vi "Check Close.vi"(8 "error in (no error)":errorcluster, 11 "Module in":refnum<class "Module.lvclass">) -> (0 "error out":errorcluster, 2 "Stop":bool, 3 "Module out":refnum<class "Module.lvclass">)   [LabVIEW 2020, in "Volatus.lvlib" / "Module.lvclass"]
uses:
  Module.lvclass
  Module.lvclass/Module.ctl
  Event Level.ctl
  State.ctl
  8a5c0d25-5ba7-4b78-9c46-4168992e23e7.vi
  Volatus.lvlib
panel:
  out "Module ID":string
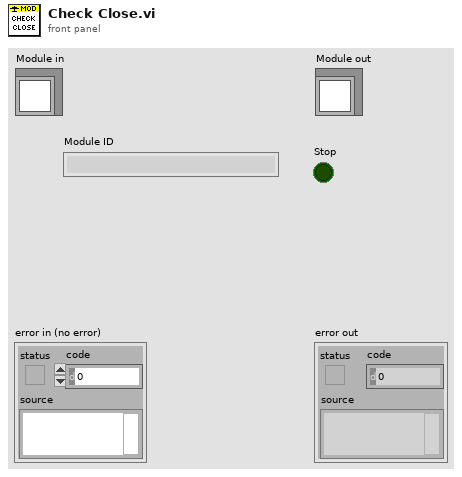
[diagram p1: front panel]
types:
  T1 = typedef "Volatus.lvlib/Module.lvclass/State.ctl" = enum16{"Unknown", "Launched", "Starting", "Running", "Stopping", "Stopped", "Error - Starting", "Error - Run", "Error - Stopping"}
  T2 = typedef "Volatus.lvlib/Event Level.ctl" = enum16{"Debug", "Info", "Warning", "Error"}
  T3 = typedef "Volatus.lvlib/Module Status.ctl" = cluster{"MessageQ":refnum<class "MessageQ.lvclass">, "State":T1, "Hierarchy":string[], "Forwarded":bool}
  T4 = cluster{"MsgQ":refnum<class "MessageQ.lvclass">, "Status":T3}[]
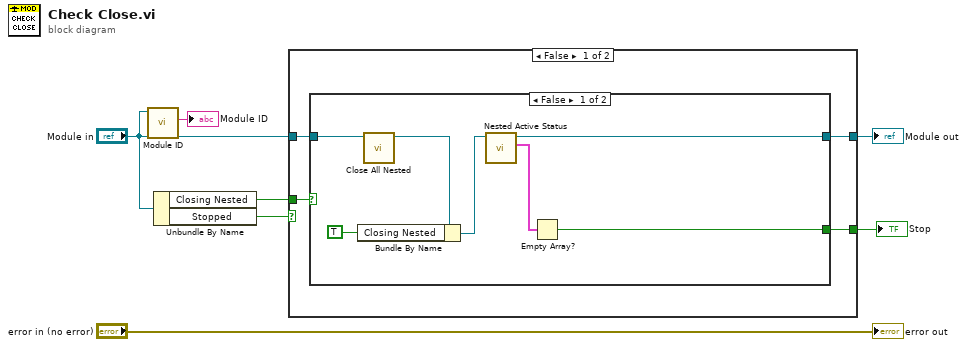
[diagram p0: block diagram]
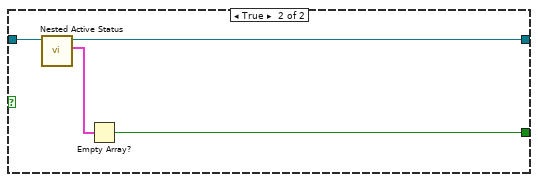
[diagram p2: hidden frame]
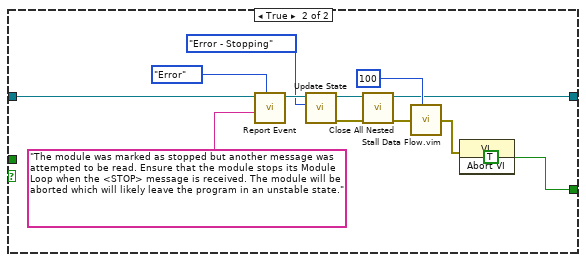
[diagram p3: hidden frame]
diagram:
  n1 = call-dynamic "Module ID.vi"("Module in"="Module in") -> ("Module ID"=→"Module ID":string)  [unwired: 10 in]
  n2 = Unbundle By Name("Module in") -> ("Closing Nested"=w7:bool, "Stopped"=w3:bool)
  n3 = case shown="False" w3 {
    tunnel: "Module in" -> [w11 w34]
    tunnel: w7 -> [w10 _]
    tunnel: [w9 w23] -> w6
    tunnel: [w8 TRUE] -> w4
    frame False {
      n4 = case shown="False" w10 {
        tunnel: w11 -> [w18 w22]
        tunnel: [w12 w21] -> w9
        tunnel: [w13 w19] -> w8
        frame False {
          n5 = call "Close All Nested.vi"("Module in"=w18) -> ("Module out"=w17:refnum<class "Module.lvclass">)  [unwired: 9 in, 1 out]
          n6 = Bundle By Name(cluster=w17, "Closing Nested"=TRUE) -> (w16:refnum<class "Module.lvclass">)
          n7 = call "Nested Active Status.vi"("Module in"=w16) -> ("Active Nested"=w14:T4, "Module out"=w12:refnum<class "Module.lvclass">)  [unwired: 7 in, 2 out]
          n8 = Empty Array?(array=w14) -> (empty?=w13:bool)
        }
        frame True {
          n9 = call "Nested Active Status.vi"("Module in"=w22) -> ("Active Nested"=w20:T4, "Module out"=w21:refnum<class "Module.lvclass">)  [unwired: 7 in, 2 out]
          n10 = Empty Array?(array=w20) -> (empty?=w19:bool)
        }
      }
    }
    frame True {
      n11 = call "Report Event.vi"("Level (Info)"=Event_Level."Error", "Message"="The module was marked as stopped but another message was attempted to be read. Ensure that the module stops its Module Loop when the <STOP> message is received. The module will be aborted which will likely leave the program in an unstable state.", "Module in"=w34) -> ("Module out"=w31:refnum<class "Module.lvclass">)  [unwired: 7 in, 1 out]
      n12 = call "Update State.vi"("State"=State."Error - Stopping", "Module in"=w31) -> ("error out"=w27:errorcluster, "Module out"=w24:refnum<class "Module.lvclass">)  [unwired: 8 in]
      n13 = call "Close All Nested.vi"("error in (no error)"=w27, "Module in"=w24) -> ("error out"=w25:errorcluster, "Module out"=w23:refnum<class "Module.lvclass">)  [unwired: 8 in]
      n14 = call "Stall Data Flow.vim"("value in"=w25, "milliseconds to wait"=u32 100) -> ("value out"=w26:errorcluster)  [unwired: 1 out]
      n15 = invoke class="VI" method="Abort VI"(error in=w26) -> ()  [unwired: 2 in, 3 out]
    }
  }
  "Module out" <- w6
  "Stop" <- w4
  "error out" <- "error in (no error)"
